vi "AU004_Schritt.vi"(10 "StateIn":dbl[](array[numeric])=[0.0, 0.0, 0.0, 0.0, 0.0, 0.0, 0.0, 0.0, 0.0, 0.0, 0.0, 0.0, 0.0, 0.0, 0.0, 0.0], 11 "Parameters":dbl[](array[numeric])=[0.05, 100.0, 1.0, 1.0, 0.0, 0.0, 0.0, 3.0, 3.0, 30.0, 1.0]) -> (2 "Values":dbl[](array[numeric]), 3 "StateOut":dbl[](array[numeric]))   [LabVIEW 2026]
doc: "AT1B virtual sensor workbench: deterministic model step. Explicit state, no hardware access. See model contract and assumptions."
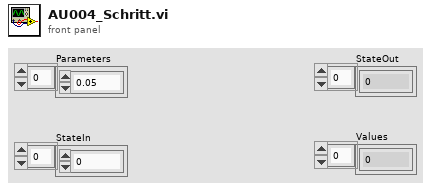
[diagram p1: front panel]
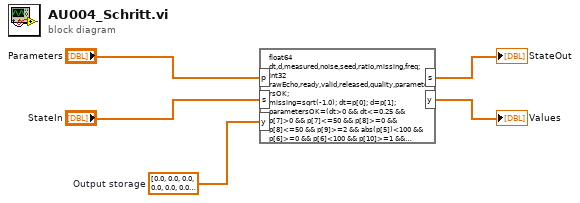
[diagram p0: block diagram]
diagram:
  w3 = dbl[] [0.0, 0.0, 0.0, 0.0, 0.0, 0.0, 0.0, 0.0, 0.0, 0.0, 0.0, 0.0, 0.0, 0.0, 0.0]  # Output storage
  n1 = formula code="float64 dt,d,measured,noise,seed,ratio,missing,freq;\nint32 rawEcho,ready,valid,released,quality,parametersOK;\nmissing=sqrt(-1.0); dt=p[0]; d=p[1];\nparametersOK=(dt>0 && dt<=0.25 && p[7]>0 && p[7]<=50 && p[8]>=0 && p[8]<=50 && p[9]>=2 && abs(p[5])<100 && p[6]>=0 && p[6]<100 && p[10]>=1 && p[10]<=2147483646);\nif(s[0]==0){s[0]=1; s[15]=p[10];}\nif(parametersOK){\n  s[13]=s[13]+dt; s[12]=s[12]-dt; if(s[12]<0){s[12]=0;}\n  seed=s[15]*16807; seed=seed-floor(seed/2147483647)*2147483647; s[15]=seed;\n  noise=p[6]*(2*seed/2147483647-1);\n  if(p[3]==0){s[9]=0; s[4]=0; s[5]=0; s[10]=0;}\n  else {s[9]=s[9]+dt;}\n  rawEcho=(p[2]>0 && d>=50 && d<=400); ready=(p[3]>0 && s[9]>=0.3);\n  released=(p[4]==0 && s[6]>0);\n  if(ready){\n    if(p[4]>0){s[5]=s[5]+dt; s[11]=0;}\n    else {\n      if(released){\n        if(s[5]>6){s[7]=1-s[7]; s[4]=0; s[12]=0.5; s[14]=12;}\n        else {if(s[5]>=2){s[4]=1; s[11]=0;}\n          else {if(s[5]>=0.7 && s[5]<=1.5){\n            if(s[4]==1){\n              if(rawEcho==0){s[8]=0; s[1]=0; s[2]=0; s[7]=0; s[4]=0; s[12]=0.5; s[14]=4;}\n              else {if(d>50){s[3]=d; s[4]=2; s[11]=0;} else {s[4]=0;}}\n            } else {if(s[4]==2){\n              if(rawEcho && s[3]>=d){s[1]=s[3]; s[2]=d; s[8]=1; s[12]=0.5; s[14]=4;}\n              s[4]=0;\n            }}\n          }}\n        }\n        s[5]=0;\n      }\n      if(s[4]>0){s[11]=s[11]+dt; if(s[11]>p[9]){s[4]=0;}}\n    }\n  }\n  s[6]=(p[4]>0);\n  quality=0; if(s[8]==0){quality=1;} if(d<50 || d>400){quality=2;} if(p[2]==0){quality=3;} if(ready==0){quality=4;} if(p[3]==0){quality=5;}\n  valid=(quality==0);\n  measured=50+floor((d+p[5]+noise-50)/p[7]+0.5)*p[7]; if(measured<50){measured=50;} if(measured>400){measured=400;}\n  y[0]=missing; y[1]=missing; y[2]=missing; y[3]=0;\n  if(valid){\n    ratio=(measured-50)/(s[1]-50); if(ratio<0){ratio=0;} if(ratio>1){ratio=1;}\n    y[0]=4+16*ratio; y[1]=50+350*ratio; y[2]=measured;\n    if(s[1]>s[2]){s[10]=(measured>=s[2] && measured<=s[1]);}\n    else {if(measured<=s[1]){s[10]=1;} if(measured>s[1]+p[8]){s[10]=0;}}\n    y[3]=s[10]; if(s[7]>0){y[3]=1-y[3];}\n  }\n  freq=0; if(s[4]==1){freq=1;} if(s[4]==2){freq=2.5;} if(s[12]>0){freq=s[14];}\n  y[4]=(rawEcho && ready); y[5]=quality; y[6]=s[4]; y[7]=s[5]; y[8]=freq;\n} else {y[0]=missing; y[1]=missing; y[2]=missing; y[3]=0; y[4]=0; y[5]=9; y[6]=s[4]; y[7]=s[5]; y[8]=0;}\ny[9]=s[8]; y[10]=s[1]; y[11]=s[2]; y[12]=s[7]; y[13]=s[13];\ny[14]=0; if(p[3]>0 && y[8]>0){ratio=s[13]*y[8]; y[14]=(ratio-floor(ratio)<0.5);}"("p"="Parameters", "s"="StateIn", "y"=w3) -> ("s"=→"StateOut":dbl[], "y"=→"Values":dbl[])
